vi "Pump Load Ctrl.vi"(8 "error in":errorcluster, 11 "Water Tunnel Results in":refnum<class "Water Tunnel Results.lvclass">) -> (0 "error out":errorcluster, 1 "Pump Load":dbl, 2 "Pump Inv U":dbl, 3 "Water Tunnel Results out":refnum<class "Water Tunnel Results.lvclass">, 4 "Water Flow":dbl)   [LabVIEW 2019, in "Results.lvlib" / "Water Tunnel Results.lvclass"]
uses:
  Water Tunnel Results.lvclass
  Water Tunnel Results.lvclass/Water Tunnel Results.ctl
  <vilib>/ErrorRing/Error Ring.xnode
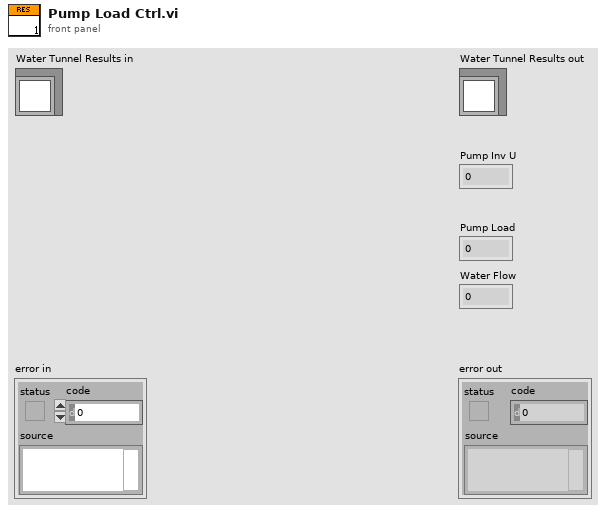
[diagram p1: front panel]
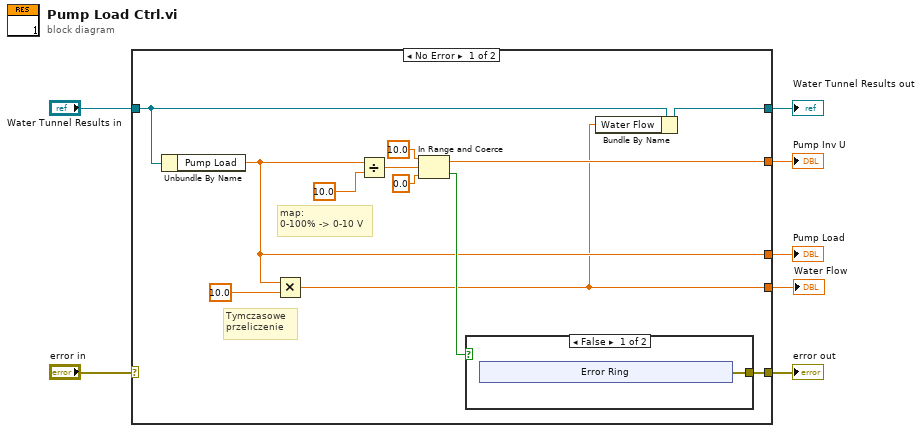
[diagram p0: block diagram]
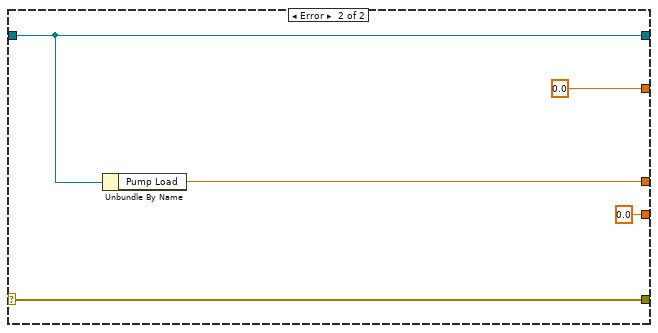
[diagram p3: hidden frame]
diagram:
  n1 = case shown="No Error" "error in" {
    selector: "error in" -> [_ w26]
    tunnel: [w12 w26] -> w6
    tunnel: [w9 w24] -> w4
    tunnel: "Water Tunnel Results in" -> [w19 w24]
    tunnel: [w14 0.0 ("upper limit")] -> w3
    tunnel: [w11 w23] -> w2
    tunnel: [w8 0.0] -> w1
    frame No Error {
      # "Tymczasowe \nprzeliczenie"
      # "map:\n0-100% -> 0-10 V"
      n2 = Unbundle By Name(w19) -> ("Pump Load"=w11:dbl)
      n3 = Multiply(x=w11, y=10.0) -> (x*y=w8:dbl)
      n4 = Divide(x=w11, y=10.0) -> (x/y=w17:dbl)
      n5 = In Range and Coerce(upper limit=10.0, x=w17, lower limit=0.0) -> (coerced(x)=w14:dbl, In Range?=w13:bool)
      n6 = case shown="False" w13 {
        tunnel: [w20 _] -> w12
        frame False {
          n7 = xnode "Error Ring"() -> ("error out"=w20:errorcluster)
        }
        frame True {
        }
      }
      n8 = Bundle By Name(cluster=w19, "Water Flow"=w8) -> (w9:refnum<class "Water Tunnel Results.lvclass">)
    }
    frame Error {
      n9 = Unbundle By Name(w24) -> ("Pump Load"=w23:dbl)
    }
  }
  "error out" <- w6
  "Water Tunnel Results out" <- w4
  "Pump Inv U" <- w3
  "Pump Load" <- w2
  "Water Flow" <- w1
